vi "template_Job_Static_VI_Reference.vi"() -> ()   [LabVIEW 2013]
doc: "Basic Job with Standard Input and Output + Job class instance"
uses:
  Job/Job.lvclass
  Job/Job.lvclass/Job.ctl
  Job/Read Abort Notifier.vi
  <vilib>/Utility/error.llb/Error Cluster From Error Code.vi
panel:
  out "Job out":refnum<class "Job.lvclass">
  out "error out":errorcluster
  in  "Job":refnum<class "Job.lvclass">
  out "stdout":string
  in  "stdin":string
  # "All Controls and Indicators are optional and do not need to be connected to the ConPane\n\n\n-- \"Job\" class input allows to monitor the Abort notifications from scheduler.\n-- \"Job\" class output allows to insert key-value pairs into data map.\n-- stdin allows to pass in commands into the job\n-- stdout allows to send back a response to the scheduler after execution completes\n-- error output terminal returns the exception code to the scheduler\n-- stdin and stdout are default labels. If they are to be named differently, one must configure the constructor node declaring the Static VI refnum."
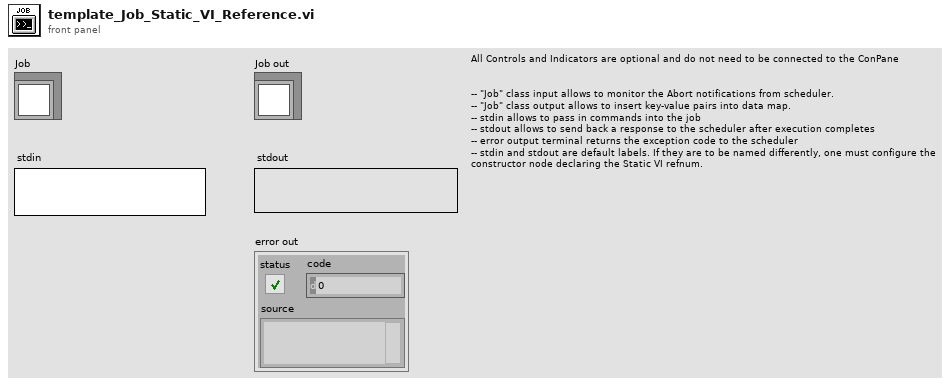
[diagram p1: front panel]
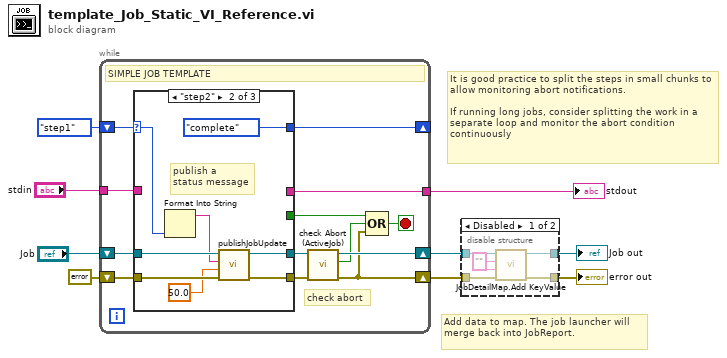
[diagram p0: block diagram]
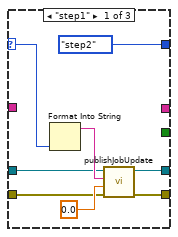
[diagram p3: hidden frame]
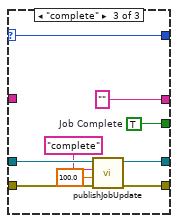
[diagram p4: hidden frame]
diagram:
  # "It is good practice to split the steps in small chunks to allow monitoring abort notifications.\n\nIf running long jobs, consider splitting the work in a separate loop and monitor the abort condition continuously"
  # "Add data to map. The job launcher will merge back into JobReport."
  n1 = while {
    tunnel: [w10] -> w4
    shift-right: [w20] -> w5
    shift-left: errorcluster {"status"=FALSE, "code"=0, "source"=""} ("error out") -> [w15]
    shift-right: [w21] -> w6
    shift-left: "Job" -> [w16]
    tunnel: "stdin" -> [w13]
    shift-right: [w11] -> _
    shift-left: enum16{"step1", "step2", "complete"}."step1" -> [w12]
    stop <- w22 stop-if-true
    # "check abort"
    # "SIMPLE JOB TEMPLATE"
    n2 = case shown="\"step2\"" w12 {
      selector: w12 -> [w27 w33 w46]
      tunnel: [_ _ w47] -> w18
      tunnel: [w25 w34 w43] -> w17
      tunnel: w16 -> [w26 w35 w44]
      tunnel: w15 -> [w23 w37 w42]
      tunnel: [w24 w36 w41] -> w14
      tunnel: w13 -> [_ _ _]
      tunnel: [enum16{"step1", "step2", "complete"}."step2" enum16{"step1", "step2", "complete"}."complete" w46] -> w11
      tunnel: [_ _ ""] -> w10
      frame "step1" {
        n3 = Format Into String(w27) -> (resulting string=w29:string)  [unwired: 3 in, 1 out]
        n4 = call "publishJobUpdate.vi"("error in (no error)"=w23, "% Complete (NaN if unknown)"=0.0, "Status Message"=w29, "Job in"=w26) -> ("error out"=w24:errorcluster, "Job out"=w25:refnum<class "Job.lvclass">)  [unwired: 6 in]
      }
      frame "step2" {
        # "publish a\nstatus message"
        n5 = Format Into String(w33) -> (resulting string=w32:string)  [unwired: 3 in, 1 out]
        n6 = call "publishJobUpdate.vi"("error in (no error)"=w37, "% Complete (NaN if unknown)"=50.0, "Status Message"=w32, "Job in"=w35) -> ("error out"=w36:errorcluster, "Job out"=w34:refnum<class "Job.lvclass">)  [unwired: 6 in]
      }
      frame "complete" {
        w47 = TRUE  # Job Complete
        n7 = call "publishJobUpdate.vi"("error in (no error)"=w42, "% Complete (NaN if unknown)"=100.0, "Status Message"="complete", "Job in"=w44) -> ("error out"=w41:errorcluster, "Job out"=w43:refnum<class "Job.lvclass">)  [unwired: 6 in]
      }
    }
    n8 = call "check Abort (ActiveJob).vi"("error in (no error)"=w14, "Job in"=w17) -> ("error out"=w20:errorcluster, "Abort"=w19:bool, "Job out"=w21:refnum<class "Job.lvclass">)  [unwired: 6 in, 1 out]
    n9 = Compound Arithmetic op=OR(w18, w19, w20) -> (w22:bool)
  }
  "stdout" <- w4
  n10 = disable-structure shown="Disabled" {
    disable-tunnel: [w52 w54] -> w9
    disable-tunnel: [w51 w53] -> w8
    disable-tunnel: w6 -> [w50 w54]
    disable-tunnel: w5 -> [w49 w53]
    frame Disabled {
      w48 = "" ("Key")
      n11 = call "JobDetailMap.Add KeyValue.vi"("error in (no error)"=w49, "Value"=w48, "Key"=w48, "Job in"=w50) -> ("error out"=w51:errorcluster, "Job out"=w52:refnum<class "Job.lvclass">)  [unwired: 6 in]
    }
    frame Enabled {
    }
  }
  "error out" <- w8
  "Job out" <- w9
